vi "Initialize.vi"(6 "Filter":T1 {"Deny List (ID)" format="%.0x"; "Allow List (ID)" format="%.0x"}, 7 "Use OS Timestamp":bool, 8 "error in (no error)":errorcluster, 9 "Port Configuration":T2={"Mode"=enum."CAN FD", "Baud Rate"=500000, "Temination On"=TRUE, "Subordinate"=FALSE, "Echo TX"=FALSE, "FD Config"={"FD Baud Rate"=2000000, "ISO Mode"=TRUE, "BRS Enabled"=TRUE}} {"FD Config"."FD Baud Rate" format="%.0p"; "Baud Rate" format="%.0p"}, 10 "Interface":string, 11 "CANsub_CAN_RW in":refnum<class "CAN RW CANsub.lvclass">) -> (0 "error out":errorcluster, 3 "CANsub_CAN_RW out":refnum<class "CAN RW CANsub.lvclass">)   [LabVIEW 2021, in "CAN RW CANsub.lvclass"]
doc: "Prepares the object for one CANsub channel. Interface is <host>/<channel>, for example 192.168.0.49/2. Makes the API channel object and all buffers. Does not use the network: call Start Reader or Start Writer to open the channel. Setup/teardown only: do not call in a periodic loop (allocates)."
uses:
  CAN RW CANsub.lvclass
  C:/Program Files/National Instruments/LabVIEW 2025/vi.lib/CIF Foundation/CIF CAN RW Core/CAN_RW_CORE.lvclass
  CAN RW CANsub.lvclass/CAN RW CANsub.ctl
  <vilib>/CIF Foundation/CIF CAN RW Core/CAN_RW_CORE.lvclass
  CANsub/c_client/api/CANsub_Channel/CANsub_Channel.lvclass
  CANsub/c_client/api/Pcap/CANsub_Pcap_Options.ctl
  CANsub/c_client/api/CANsub_API.lvlib
  <vilib>/CIF Foundation/CIF CAN RW Core/typedef/CAN Mode.ctl
  <vilib>/CIF Foundation/CIF CAN RW Core/typedef/FD Config.ctl
  <vilib>/CIF Foundation/CIF CAN RW Core/typedef/CAN Port Configuration.ctl
  <vilib>/CIF Foundation/CIF CAN RW Core/typedef/CAN Filter.ctl
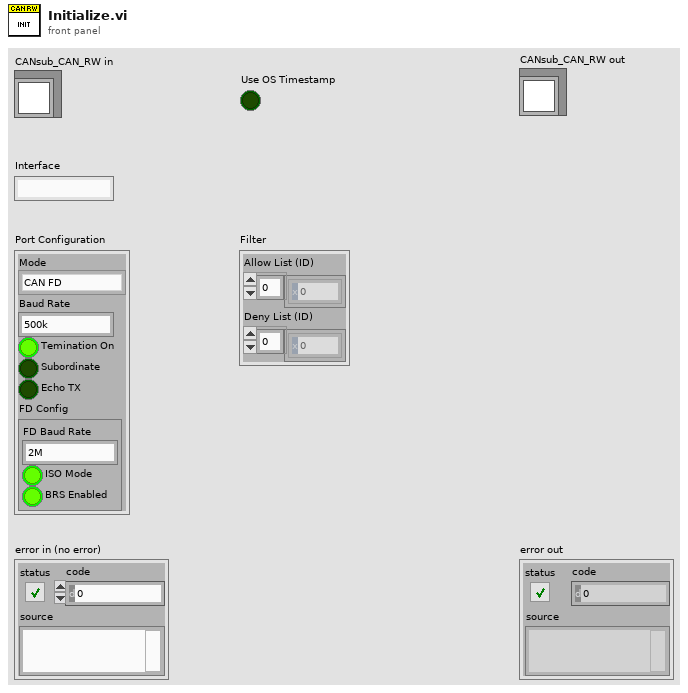
[diagram p1: front panel]
types:
  T1 = typedef "CAN_RW_CORE.lvclass/CAN Filter.ctl" = cluster{"Allow List (ID)":u32[], "Deny List (ID)":u32[]}
  T2 = typedef "CAN_RW_CORE.lvclass/CAN Port Configuration.ctl" = cluster{"Mode":T3, "Baud Rate":u64, "Temination On":bool, "Subordinate":bool, "Echo TX":bool, "FD Config":T4}
  T3 = typedef "CAN_RW_CORE.lvclass/CAN Mode.ctl" = enum16{"CAN 2.0", "CAN FD"}
  T4 = typedef "CAN_RW_CORE.lvclass/FD Config.ctl" = cluster{"FD Baud Rate":u64, "ISO Mode":bool, "BRS Enabled":bool}
  T5 = typedef "CANsub_API.lvlib/CANsub_Pcap_Options.ctl" = cluster{"allow list":u32[], "deny list":u32[], "TAI minus UTC (s)":i32, "keep TX acks":bool, "little endian":bool}
  T6 = typedef "CANsub_API.lvlib/CANsub_Config.ctl" = cluster{"connection":T7, "bit rates":T8, "listen only":bool, "filters":T9[], "read mode":T10, "max bytes per read":i32, "reader FIFO depth":i32, "reader priority":i32, "ownership":T11}
  T7 = typedef "CANsub_Common.lvlib/CANsub_connection.ctl" = cluster{"host":string, "channel":u8, "cert path":path}
  T8 = typedef "CANsub_Common.lvlib/CANsub_Bit_Rates.ctl" = cluster{"nominal bit rate":u32, "nominal sample point":dbl, "data bit rate":u32, "data sample point":dbl}
  T9 = typedef "CANsub_API.lvlib/CANsub_Filter.ctl" = cluster{"extended":bool, "range":bool, "f1":u32, "f2":u32}
  T10 = typedef "CANsub_API.lvlib/CANsub_Read_Mode.ctl" = enum16{"Poll", "Reader"}
  T11 = typedef "CANsub_API.lvlib/CANsub_Ownership.ctl" = enum16{"Direct", "Shared"}
  T12 = typedef "CANsub_API.lvlib/CANsub_Frames.ctl" = cluster{"count":i32, "t_dev":dbl[], "id":u32[], "flags":u16[], "dlc":u8[], "data len":u8[], "data":u8[]}
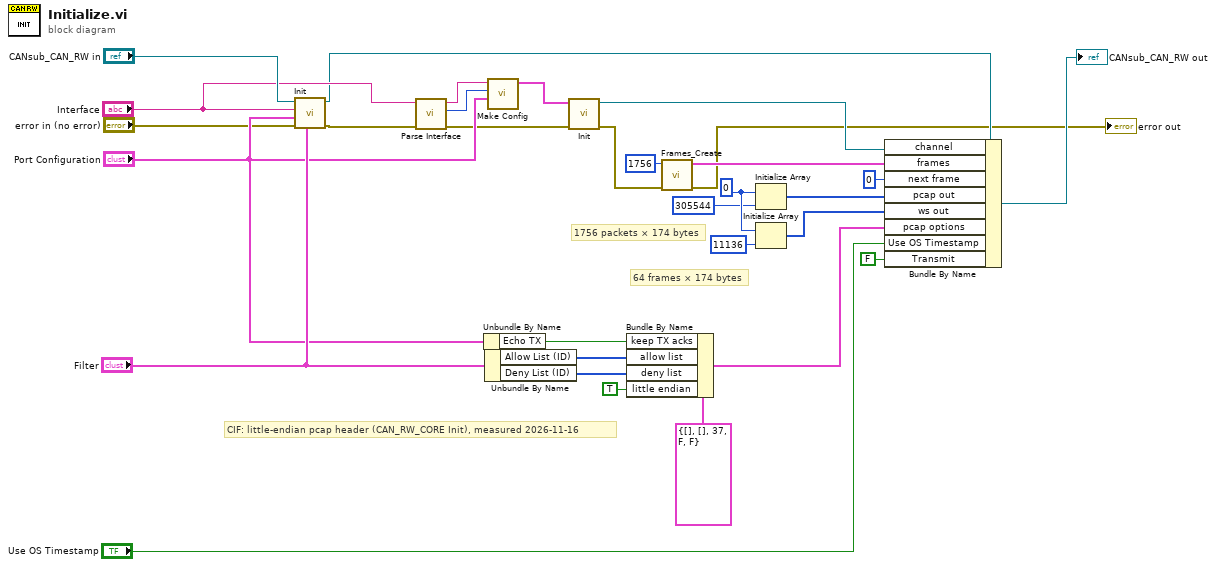
[diagram p0: block diagram]
diagram:
  w25 = u8 0
  # "CIF: little-endian pcap header (CAN_RW_CORE Init), measured 2026-11-16"
  # "1756 packets × 174 bytes"
  # "64 frames × 174 bytes"
  n1 = call <vilib>:"Init.vi"("Filter"="Filter", "error in (no error)"="error in (no error)", "Port Configuration"="Port Configuration", "Interface"="Interface", "CAN_RW_CORE in"="CANsub_CAN_RW in") -> ("error out"=w5:errorcluster, "CAN_RW_CORE out"=w15:refnum<class "CAN RW CANsub.lvclass">)  [unwired: 5 in]
  n2 = call "Parse Interface.vi"("error in (no error)"=w5, "Interface"="Interface") -> ("error out"=w4:errorcluster, "channel"=w28:u8, "host"=w29:string)  [unwired: 7 in]
  n3 = Unbundle By Name("Port Configuration") -> ("Echo TX"=w18:bool)
  n4 = Unbundle By Name("Filter") -> ("Allow List (ID)"=w17:u32[], "Deny List (ID)"=w16:u32[])
  n5 = call "Make Config.vi"("Port Configuration"="Port Configuration", "channel"=w28, "host"=w29) -> ("config"=w27:T6)  [unwired: 8 in]
  n6 = call <vilib>:"Init.vi"("error in (no error)"=w4, "config"=w27) -> ("error out"=w2:errorcluster, "channel out"=w6:refnum<class "CANsub_Channel.lvclass">)  [unwired: 7 in, 1 out]
  n7 = Bundle By Name(cluster=T5 {"allow list"=[], "deny list"=[], "TAI minus UTC (s)"=37, "keep TX acks"=FALSE, "little endian"=FALSE} ("CANsub_Pcap_Options"), "keep TX acks"=w18, "allow list"=w17, "deny list"=w16, "little endian"=TRUE) -> (w13:T5)
  n8 = call "Frames_Create.vi"("error in (no error)"=w2, "capacity"=1756) -> ("error out"=→"error out":errorcluster, "frames"=w7:T12)  [unwired: 8 in]
  n9 = Initialize Array(w25, 305544 ("dimension size")) -> (w9:u8[])
  n10 = Initialize Array(w25, 11136 ("dimension size")) -> (w10:u8[])
  n11 = Bundle By Name(cluster=w15, "channel"=w6, "frames"=w7, "next frame"=0, "pcap out"=w9, "ws out"=w10, "pcap options"=w13, "Use OS Timestamp"="Use OS Timestamp", "Transmit"=FALSE) -> (→"CANsub_CAN_RW out":refnum<class "CAN RW CANsub.lvclass">)
